vi "Change Port.vi"   [LabVIEW 2023]
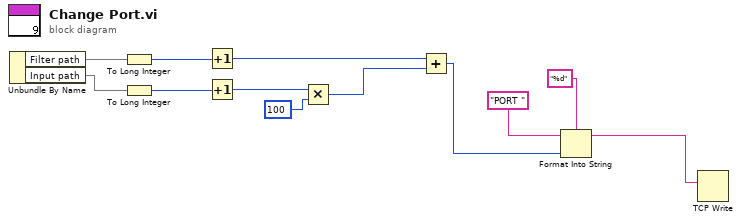
[diagram p0: block diagram]
diagram:
  n1 = Unbundle By Name() -> ("Filter path"=w10, "Input path"=w13)  [unwired: 1 in]
  n2 = To Long Integer(number=w10) -> (32bit integer=w11:i32)
  n3 = To Long Integer(number=w13) -> (32bit integer=w12:i32)
  n4 = Increment(x=w11) -> (x+1=w7:i32)
  n5 = Increment(x=w12) -> (x+1=w9:i32)
  n6 = Multiply(x=w9, y=100) -> (x*y=w6:i32)
  n7 = Add(x=w7, y=w6) -> (x+y=w3:i32)
  n8 = Format Into String(format string="%d" ("포맷 문자열"), initial string="PORT " ("초기 문자열"), w3) -> (resulting string=w2:string, error out=w1:errorcluster)  [unwired: 1 in]
  n9 = TCP Write(data in=w2) -> ()  [unwired: 3 in, 3 out]
